vi "Reserve Registered Sessions.vi"(6 "timeout (ms)":i32=10000, 8 "error in":errorcluster, 9 "instrument type id":string) -> (0 "error out":errorcluster, 3 "session reservation out":refnum<class "Session Reservation.lvclass">)   [LabVIEW 2021, in "NI Session Management V1 Client.lvlib" / "Session Reservation.lvclass"]
doc: "Reserves all registered session(s) with the specified <b>instrument type id</b>. If the <b>instrument type id</b> is an empty string, reserves all registered sessions for all instrument types."
uses:
  Session Reservation.lvclass
  Session Reservation.lvclass/Session Reservation.ctl
  gRPC/Generated APIs/ni/measurementlink/sessionmanagement/v1/RPC Messages/ni_measurementlink_sessionmanagement_v1_ReserveAllRegisteredSessionsRequest.ctl
  gRPC/Generated APIs/ni/measurementlink/sessionmanagement/v1/ni.measurementlink.sessionmanagement.v1.api.lvlib
  gRPC/Generated APIs/ni/measurementlink/sessionmanagement/v1/RPC Messages/ni_measurementlink_PinMapContext.ctl
  IReservation Observer/IReservation Observer.lvclass
  gRPC/Generated APIs/ni/measurementlink/sessionmanagement/v1/RPC Messages/nidevice_grpc_Session.ctl
  gRPC/Generated APIs/ni/measurementlink/sessionmanagement/v1/RPC Messages/ni_measurementlink_sessionmanagement_v1_ChannelMapping.ctl
  gRPC/Generated APIs/ni/measurementlink/sessionmanagement/v1/RPC Messages/ni_measurementlink_sessionmanagement_v1_SessionInformation.ctl
  gRPC/Generated APIs/ni/measurementlink/sessionmanagement/v1/RPC Messages/ni_measurementlink_sessionmanagement_v1_MultiplexerSessionInformation.ctl
  gRPC/Generated APIs/ni/measurementlink/sessionmanagement/v1/RPC Messages/ni_measurementlink_sessionmanagement_v1_ResolvedPinsOrRelays.ctl
  gRPC/Generated APIs/ni/measurementlink/sessionmanagement/v1/RPC Messages/ni_measurementlink_sessionmanagement_v1_ReserveSessionsResponse_GroupMappingsEntry.ctl
  gRPC/Generated APIs/ni/measurementlink/sessionmanagement/v1/RPC Messages/ni_measurementlink_sessionmanagement_v1_ReserveSessionsResponse.ctl
  gRPC/Generated APIs/ni/measurementlink/sessionmanagement/v1/RPC Messages/ni_measurementlink_sessionmanagement_v1_ReserveAllRegisteredSessionsRequest_AnnotationsEntry.ctl
  gRPC/Generated APIs/ni/measurementlink/sessionmanagement/v1/RPC Messages/ni_measurementlink_sessionmanagement_v1_SessionInformation_AnnotationsEntry.ctl
  gRPC/Generated APIs/ni/measurementlink/sessionmanagement/v1/RPC Messages/ni_measurementlink_sessionmanagement_v1_MultiplexerSessionInformation_AnnotationsEntry.ctl
  a5b56289-58b6-41e3-9e53-e8f533507d6d.vi
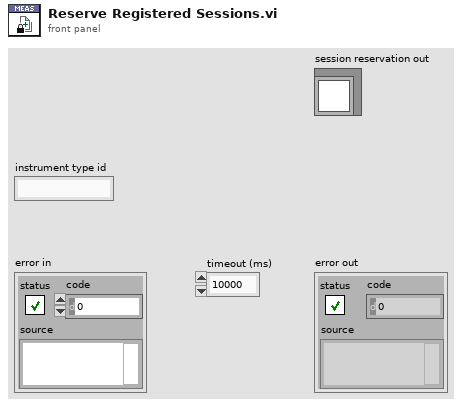
[diagram p1: front panel]
types:
  T1 = typedef "ni.measurementlink.sessionmanagement.v1.api.lvlib/ni_measurementlink_sessionmanagement_v1_ReserveAllRegisteredSessionsRequest_AnnotationsEntry.ctl" = cluster{"key":string, "value":string}
  T2 = typedef "ni.measurementlink.sessionmanagement.v1.api.lvlib/ni_measurementlink_sessionmanagement_v1_ReserveSessionsResponse.ctl" = cluster{"sessions":T3[], "multiplexer_sessions":T7[], "group_mappings":T9[]}
  T3 = typedef "ni.measurementlink.sessionmanagement.v1.api.lvlib/ni_measurementlink_sessionmanagement_v1_SessionInformation.ctl" = cluster{"session":T4, "resource_name":string, "channel_list":string, "instrument_type_id":string, "session_exists":bool, "session_reserved":bool, "channel_mappings":T5[], "annotations":T6[]}
  T4 = typedef "ni.measurementlink.sessionmanagement.v1.api.lvlib/nidevice_grpc_Session.ctl" = cluster{"name":string}
  T5 = typedef "ni.measurementlink.sessionmanagement.v1.api.lvlib/ni_measurementlink_sessionmanagement_v1_ChannelMapping.ctl" = cluster{"pin_or_relay_name":string, "site":i32, "channel":string, "multiplexer_resource_name":string, "multiplexer_route":string}
  T6 = typedef "ni.measurementlink.sessionmanagement.v1.api.lvlib/ni_measurementlink_sessionmanagement_v1_SessionInformation_AnnotationsEntry.ctl" = cluster{"key":string, "value":string}
  T7 = typedef "ni.measurementlink.sessionmanagement.v1.api.lvlib/ni_measurementlink_sessionmanagement_v1_MultiplexerSessionInformation.ctl" = cluster{"session":T4, "resource_name":string, "multiplexer_type_id":string, "session_exists":bool, "annotations":T8[]}
  T8 = typedef "ni.measurementlink.sessionmanagement.v1.api.lvlib/ni_measurementlink_sessionmanagement_v1_MultiplexerSessionInformation_AnnotationsEntry.ctl" = cluster{"key":string, "value":string}
  T9 = typedef "ni.measurementlink.sessionmanagement.v1.api.lvlib/ni_measurementlink_sessionmanagement_v1_ReserveSessionsResponse_GroupMappingsEntry.ctl" = cluster{"key":string, "value":T10}
  T10 = typedef "ni.measurementlink.sessionmanagement.v1.api.lvlib/ni_measurementlink_sessionmanagement_v1_ResolvedPinsOrRelays.ctl" = cluster{"pin_or_relay_names":string[]}
  T11 = typedef "ni.measurementlink.sessionmanagement.v1.api.lvlib/ni_measurementlink_PinMapContext.ctl" = cluster{"pin_map_id":string, "sites":i32[]}
  T12 = typedef "ni.measurementlink.sessionmanagement.v1.api.lvlib/ni_measurementlink_sessionmanagement_v1_ReserveAllRegisteredSessionsRequest.ctl" = cluster{"timeout_in_milliseconds":i32, "instrument_type_id":string, "annotations":T1[]}
  T13 = typedef "ni.measurementlink.sessionmanagement.v1.api.lvlib/ni_measurementlink_sessionmanagement_v1_ReserveAllRegisteredSessionsResponse.ctl" = cluster{"sessions":T3[]}
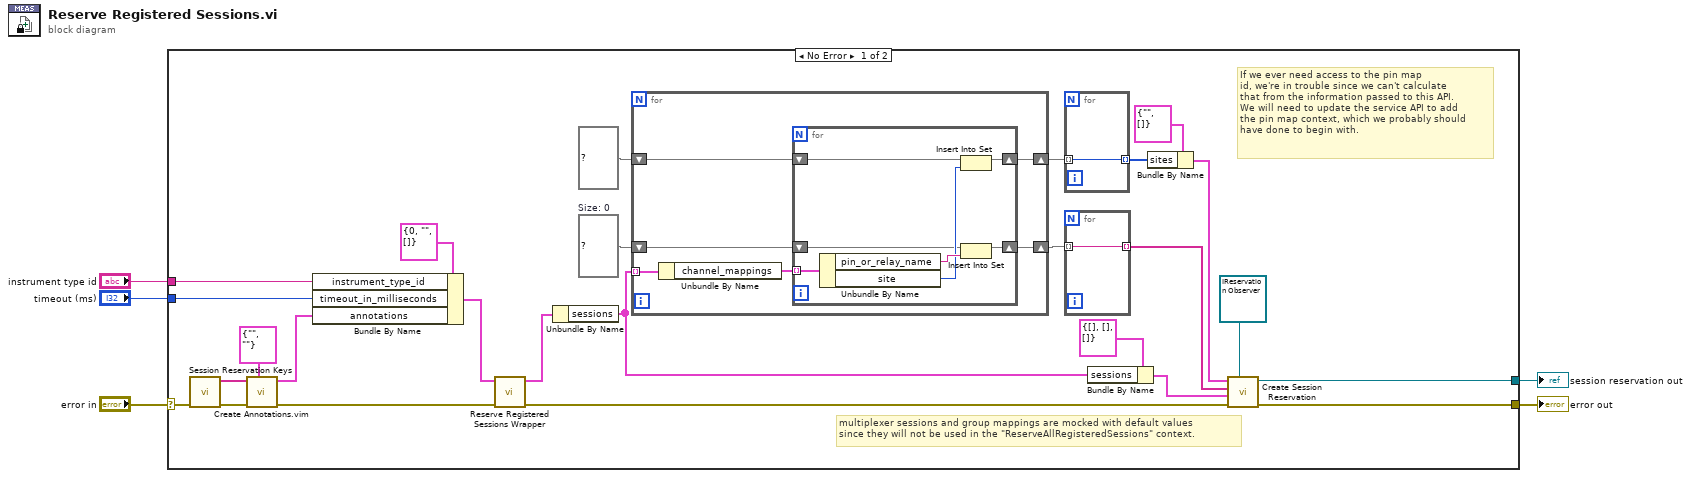
[diagram p0: block diagram]
diagram:
  n1 = case shown="No Error" "error in" {
    selector: "error in" -> [w13 w46]
    tunnel: [w29 _] -> w4
    tunnel: [w27 w46] -> w5
    tunnel: "instrument type id" -> [w12 _]
    tunnel: "timeout (ms)" -> [w11 _]
    frame No Error {
      w24 = set{string} {}  # Size: 0
      # "multiplexer sessions and group mappings are mocked with default values\nsince they will not be used in the \"ReserveAllRegisteredSessions\" context."
      # "If we ever need access to the pin map\nid, we're in trouble since we can't calculate\nthat from the information passed to this API.\nWe will need to update the service API to add\nthe pin map context, which we probably should\nhave done to begin with."
      n2 = call "Session Reservation Keys.vi"() -> ("reserve annotation keys"=w9:string[])  [unwired: 11 in]
      n3 = call "Create Annotations.vim"("annotation typedef"=T1 {"key"="", "value"=""} ("ni_measurementlink_sessionmanagement_v1_ReserveAllRegisteredSessionsRequest_AnnotationsEntry"), "error in"=w13, "annotation keys"=w9) -> ("error out"=w10:errorcluster, "annotations array"=w8:T1[])  [unwired: 7 in]
      n4 = Bundle By Name(cluster=T12 {"timeout_in_milliseconds"=0, "instrument_type_id"="", "annotations"=[]} ("Request Data"), "instrument_type_id"=w12, "timeout_in_milliseconds"=w11, "annotations"=w8) -> (w30:T12)
      n5 = call "Reserve Registered Sessions Wrapper.vi"("error in"=w10, "request data"=w30) -> ("error out"=w28:errorcluster, "response data"=w26:T13)  [unwired: 8 in]
      n6 = Unbundle By Name(w26) -> ("sessions"=w14:T3[])
      n7 = for {
        tunnel: w14 -> [w38] mode=indexing
        shift-right: [w34] -> w23
        shift-left: w24 -> [w33]
        shift-right: [w35] -> w22
        shift-left: set{i32} {} ("set in") -> [w36]
        n8 = Unbundle By Name(w38) -> ("channel_mappings"=w37:T5[])
        n9 = for {
          tunnel: w37 -> [w45] mode=indexing
          shift-right: [w40] -> w34
          shift-left: w33 -> [w39]
          shift-right: [w41] -> w35
          shift-left: w36 -> [w42]
          n10 = Unbundle By Name(w45) -> ("pin_or_relay_name"=w44:string, "site"=w43:i32)
          n11 = Insert Into Set(10:w43, 11:w42) -> (3:w41:set{i32})  [unwired: 1 out]
          n12 = Insert Into Set(10:w44, 11:w39) -> (3:w40:set{string})  [unwired: 1 out]
        }
      }
      n13 = for {
        tunnel: [w31] -> w19 mode=indexing
        tunnel: w22 -> [w31] mode=indexing
      }
      n14 = for {
        tunnel: [w32] -> w21 mode=indexing
        tunnel: w23 -> [w32] mode=indexing
      }
      n15 = Bundle By Name(cluster=T2 {"sessions"=[], "multiplexer_sessions"=[], "group_mappings"=[]} ("session reservation response"), "sessions"=w14) -> (w15:T2)
      n16 = Bundle By Name(cluster=T11 {"pin_map_id"="", "sites"=[]} ("pin map context"), "sites"=w19) -> (w18:T11)
      n17 = call "Create Session Reservation.vi"("reservation observer"=refnum<class "IReservation Observer.lvclass"> refnum, "error in"=w28, "session reservation response"=w15, "pin or relay names"=w21, "pin map context"=w18) -> ("error out"=w27:errorcluster, "session reservation out"=w29:refnum<class "Session Reservation.lvclass">)  [unwired: 5 in]
    }
    frame Error {
    }
  }
  "error out" <- w5
  "session reservation out" <- w4
